vi "TrajectoryConfig_setKinematicsDiffDrive.vi"(6 "Use Accel":bool, 9 "DIFF_DRIVE_KINEMATICS":T1 {"TrackWidth_Meters" format="%20.4f"}, 11 "inTRAJECTORY_CONFIG":T2 {"End Velocity" format="%20.4f"; "StartVelocity" format="%20.4f"; "Max Acceleration" format="%20.4f"; "MaxVelocity" format="%20.4f"}) -> (3 "outTRAJECTORY_CONFIG":T2 {"End Velocity" format="%20.4f"; "StartVelocity" format="%20.4f"; "Max Acceleration" format="%20.4f"; "MaxVelocity" format="%20.4f"})   [LabVIEW 2019, in "Trajectory_Library.lvlib"]
doc: "Adds and enabled a differential drive kinematics constraint to ensure that no wheel velocity of a differential drive goes above the max velocity. The TrajectoryConfiguration max velocity is used for the differential drive max individual wheel velocity.\n\nParameters:\n - DiffDriveKinematics - The differential drive kinematics data structure\n - InTrajectoryConfig - The trajectory configuration data structure\n\nReturns:\n - OutTrajectoryConfig - Modified trajectory configuration data structure"
uses:
  Trajectory_Library.lvlib
  TypeDef/TRAJ_CONFIG.ctl
  TypeDef/DIFF_DRIVE_KINEMATICS.ctl
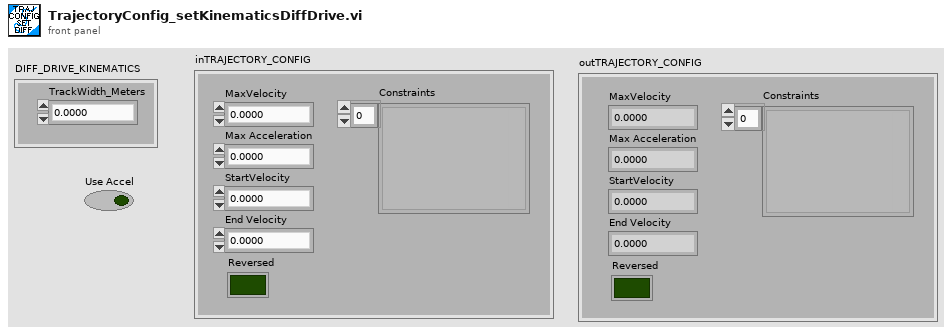
[diagram p1: front panel]
types:
  T1 = typedef "Trajectory_Library.lvlib/DIFF_DRIVE_KINEMATICS.ctl" = cluster{"TrackWidth_Meters":dbl}
  T2 = typedef "Trajectory_Library.lvlib/TRAJ_CONFIG.ctl" = cluster{"MaxVelocity":dbl, "Max Acceleration":dbl, "StartVelocity":dbl, "End Velocity":dbl, "Reversed":bool, "Constraints":variant[]}
  T3 = typedef "WPILib_Math.lvlib/TRAJ_CONSTRAINT_DIIF_DRIVE_KINEMATICS.ctl" = cluster{"Max Speed (M/S)":dbl, "DIFF_DRIVE_KINEMATICS":T4, "Max Accel (M/S2)":dbl}
  T4 = typedef "WPILib_Math.lvlib/DIFF_DRIVE_KINEMATICS.ctl" = cluster{"TrackWidth_Meters":dbl}
  T5 = typedef "WPILib_Math.lvlib/TRAJ_CONFIG.ctl" = cluster{"MaxVelocity":dbl, "Max Acceleration":dbl, "StartVelocity":dbl, "End Velocity":dbl, "Reversed":bool, "Constraints":variant[]}
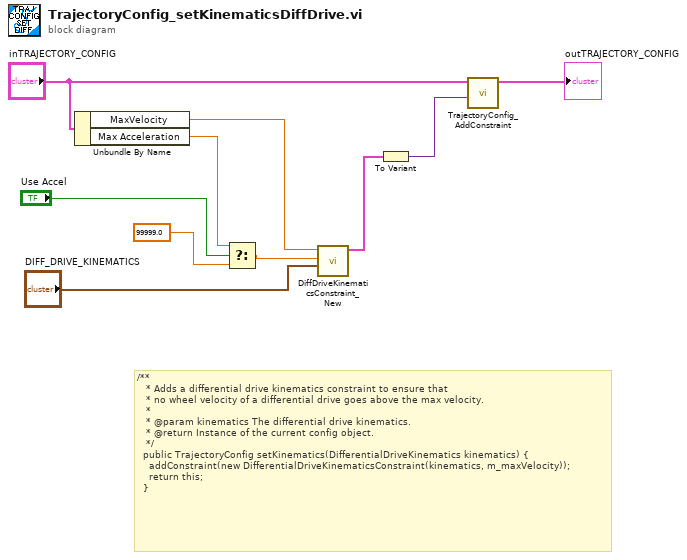
[diagram p0: block diagram]
diagram:
  # "/**\n   * Adds a differential drive kinematics constraint to ensure that\n   * no wheel velocity of a differential drive goes above the max velocity.\n   *\n   * @param kinematics The differential drive kinematics.\n   * @return Instance of the current config object.\n   */\n  public TrajectoryConfig setKinematics(DifferentialDriveKinematics kinematics) {\n    addConstraint(new DifferentialDriveKinematicsConstraint(kinematics, m_maxVelocity));\n    return this;\n  }"
  n1 = Unbundle By Name("inTRAJECTORY_CONFIG") -> ("MaxVelocity"=w10:dbl, "Max Acceleration"=w6:dbl)
  n2 = Select(t=w6, s="Use Accel", f=99999.0) -> (s? t:f=w8:dbl)
  n3 = call "DiffDriveKinematicsConstraint_New.vi"("DIFF_DRIVE_KINEMATICS"="DIFF_DRIVE_KINEMATICS", "Max Accel (M/S2)"=w8, "Max Speed (M/S)"=w10) -> ("DIFF_DRIVE_KINE_CONSTRAINT"=w2:T3)  [unwired: 8 in]
  n4 = To Variant(anything=w2) -> (Variant=w4:variant)
  n5 = call "TrajectoryConfig_AddConstraint.vi"("Constraint"=w4, "inTRAJECTORY_CONFIG"="inTRAJECTORY_CONFIG") -> ("outTRAJECTORY_CONFIG"=→"outTRAJECTORY_CONFIG":T5)  [unwired: 9 in]
